vi "Example Test JSON Schema.vi"() -> ()   [LabVIEW 2020]
uses:
  2e09bf10-32e6-4e98-8767-bf37edf36c6f.vi
  1d5c4e22-c6bb-4e91-903e-9e3f39d23dd2.vi
  <vilib>/JDP Science/JSONtext/Variant to JSON Text.vi
  <vilib>/JDP Science/JSONtext/LVClass Serializer/JSONtext LVClass Serializer.lvclass
  <vilib>/JDP Science/JSONtext/JSONtext.lvlib
panel:
  in  "strict?":bool=TRUE
  out "JSON Validated":bool
  out "Path to Failed Test":string
  out "<JSON>Failed Test":string
  out "<JSON>Failed SubJSON":string
  in  "books":T1(array[cluster])=[{"title"="book A", "time to read (hrs)"=4.5, "finished"=FALSE}, {"title"="book B", "time to read (hrs)"=4.5, "finished"=TRUE}]
  out "Serialized to JSON":string
  out "error out":errorcluster
  out "Generated JSON Schema":string
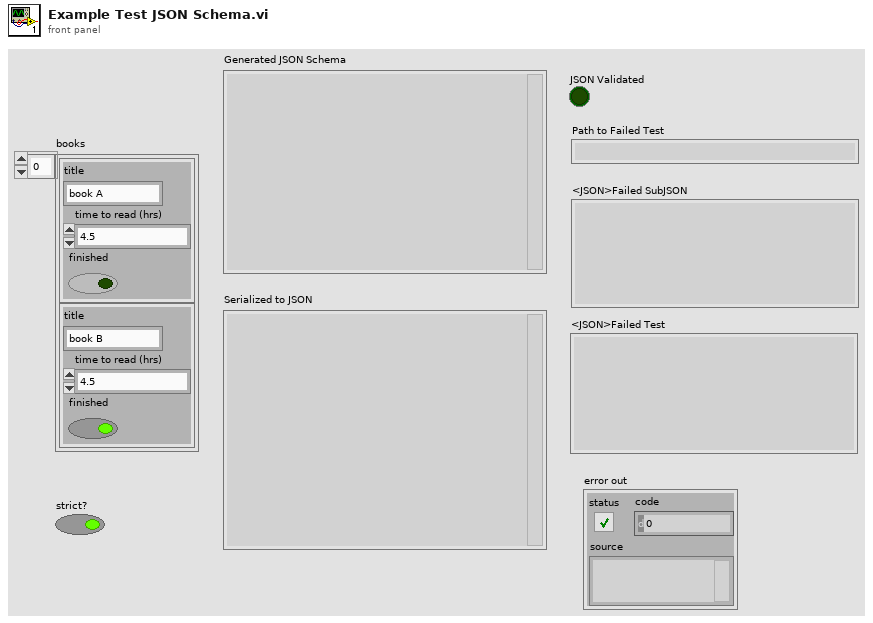
[diagram p1: front panel]
types:
  T1 = cluster{"title":string, "time to read (hrs)":dbl, "finished":bool}[]
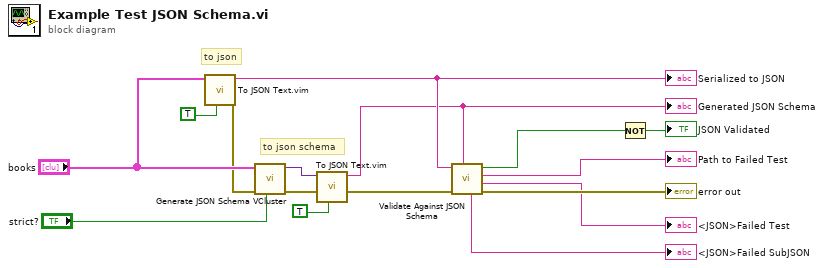
[diagram p0: block diagram]
diagram:
  # "to json"
  # "to json schema"
  n1 = call "To JSON Text.vim"("Pretty Print?"=TRUE, "Anything"="books") -> ("error out"=w3:errorcluster, "<JSON>"=w13:string)  [unwired: 8 in]
  "Serialized to JSON" <- w13
  n2 = call "Generate JSON Schema VCluster.vi"("strict?"="strict?", "error in (no error)"=w3, "type"="books") -> ("error out"=w2:errorcluster, "json schema cluster"=w16:variant)  [unwired: 7 in]
  n3 = call "To JSON Text.vim"("Pretty Print?"=TRUE, "error in (no error)"=w2, "Anything"=w16) -> ("error out"=w7:errorcluster, "<JSON>"=w12:string)  [unwired: 7 in]
  "Generated JSON Schema" <- w12
  n4 = call <vilib>:"Validate Against JSON Schema.vi"("JSON Schema"=w12, "error in (no error)"=w7, "JSON"=w13) -> ("error out"=→"error out":errorcluster, "<JSON>Failed Test"=→"<JSON>Failed Test":string, "Path to Failed Test"=→"Path to Failed Test":string, "Invalid"=w6:bool, "<JSON>Failed SubJSON"=→"<JSON>Failed SubJSON":string)  [unwired: 4 in]
  n5 = Not(x=w6) -> (.not. x?=→"JSON Validated":bool)
